vi "Get Modification Flags.vi"(8 "error in (no error)":errorcluster, 10 "Saved VI in":refnum<class "Item.lvclass">, 11 "VI in":refnum<class "VI.lvclass">) -> (0 "error out":errorcluster, 1 "Modification Flags":bool[](array[boolean]), 2 "Saved VI out":refnum<class "VI.lvclass">, 3 "VI out":refnum<class "VI.lvclass">)   [LabVIEW 2020, in "VI Properties Editor.lvlib" / "VI.lvclass"]
doc: "Gets the modification flags of <B>VI in</B> by comparing it to <B>Saved VI in</B>."
uses:
  VI.lvclass
  Item/Item.lvclass
  Control/Control.lvclass
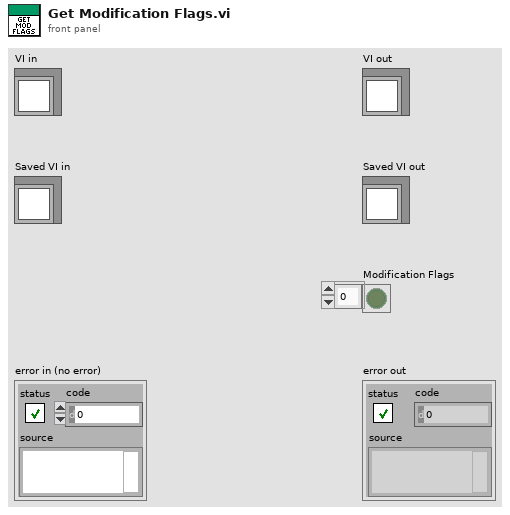
[diagram p1: front panel]
types:
  T1 = enum16{"Share clones between instances", "Preallocate clone for each instance"}
  T2 = enum32{"invalid execution system", "user interface", "standard", "instrument i/o", "data acquisition", "other 1", "other 2", "same as caller"}
  T3 = enum32{"invalid priority", "background priority", "normal priority", "above normal priority", "high priority", "time critical priority", "subroutine"}
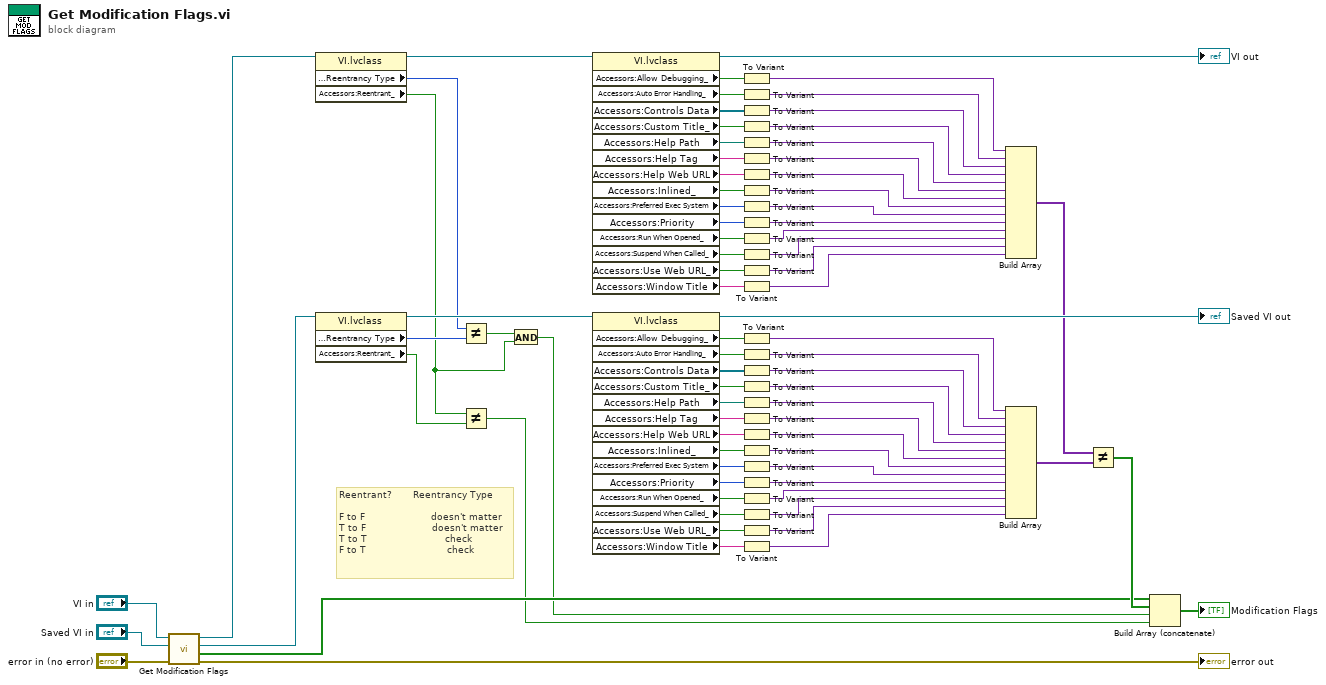
[diagram p0: block diagram]
diagram:
  # "Reentrant?       Reentrancy Type\n\nF to F                      doesn't matter\nT to F                      doesn't matter\nT to T                          check\nF to T                           check"
  n1 = call-parent "Get Modification Flags.vi"("error in (no error)"="error in (no error)", "Saved Item in"="Saved VI in", "Item in"="VI in") -> ("error out"=→"error out":errorcluster, "Modification Flags"=w13:bool[], "Saved Item out"=w10:refnum<class "VI.lvclass">, "Item out"=w8:refnum<class "VI.lvclass">)  [unwired: 5 in]
  n2 = property class="VI.lvclass"(reference=w8) -> (reference out=w9:refnum<class "VI.lvclass">, "Accessors:Reentrancy Type"=w7:T1, "Accessors:Reentrant_"=w1:bool)  [unwired: 1 in, 1 out]
  n3 = property class="VI.lvclass"(reference=w10) -> (reference out=w11:refnum<class "VI.lvclass">, "Accessors:Reentrancy Type"=w6:T1, "Accessors:Reentrant_"=w4:bool)  [unwired: 1 in, 1 out]
  n4 = Not Equal?(x=w7, y=w6) -> (x != y?=w5:bool)
  n5 = Not Equal?(x=w1, y=w4) -> (x != y?=w2:bool)
  n6 = And(x=w5, y=w1) -> (x .and. y?=w3:bool)
  n7 = property class="VI.lvclass"(reference=w9) -> (reference out=→"VI out":refnum<class "VI.lvclass">, "Accessors:Allow Debugging_"=w72:bool, "Accessors:Auto Error Handling_"=w71:bool, "Accessors:Controls Data"=w70:refnum<class "Control.lvclass">[], "Accessors:Custom Title_"=w69:bool, "Accessors:Help Path"=w68:path, "Accessors:Help Tag"=w67:string, "Accessors:Help Web URL"=w66:string, "Accessors:Inlined_"=w65:bool, "Accessors:Preferred Exec System"=w64:T2, "Accessors:Priority"=w63:T3, "Accessors:Run When Opened_"=w62:bool, "Accessors:Suspend When Called_"=w61:bool, "Accessors:Use Web URL_"=w60:bool, "Accessors:Window Title"=w59:string)  [unwired: 1 in, 1 out]
  n8 = property class="VI.lvclass"(reference=w11) -> (reference out=→"Saved VI out":refnum<class "VI.lvclass">, "Accessors:Allow Debugging_"=w16:bool, "Accessors:Auto Error Handling_"=w17:bool, "Accessors:Controls Data"=w18:refnum<class "Control.lvclass">[], "Accessors:Custom Title_"=w19:bool, "Accessors:Help Path"=w20:path, "Accessors:Help Tag"=w21:string, "Accessors:Help Web URL"=w22:string, "Accessors:Inlined_"=w23:bool, "Accessors:Preferred Exec System"=w24:T2, "Accessors:Priority"=w25:T3, "Accessors:Run When Opened_"=w26:bool, "Accessors:Suspend When Called_"=w27:bool, "Accessors:Use Web URL_"=w28:bool, "Accessors:Window Title"=w29:string)  [unwired: 1 in, 1 out]
  n9 = To Variant(anything=w72) -> (Variant=w58:variant)
  n10 = To Variant(anything=w71) -> (Variant=w57:variant)
  n11 = To Variant(anything=w70) -> (Variant=w56:variant)
  n12 = To Variant(anything=w69) -> (Variant=w55:variant)
  n13 = To Variant(anything=w68) -> (Variant=w54:variant)
  n14 = To Variant(anything=w67) -> (Variant=w53:variant)
  n15 = To Variant(anything=w66) -> (Variant=w52:variant)
  n16 = To Variant(anything=w65) -> (Variant=w51:variant)
  n17 = To Variant(anything=w64) -> (Variant=w50:variant)
  n18 = To Variant(anything=w63) -> (Variant=w49:variant)
  n19 = To Variant(anything=w62) -> (Variant=w48:variant)
  n20 = To Variant(anything=w61) -> (Variant=w47:variant)
  n21 = To Variant(anything=w60) -> (Variant=w46:variant)
  n22 = To Variant(anything=w59) -> (Variant=w45:variant)
  n23 = To Variant(anything=w16) -> (Variant=w30:variant)
  n24 = To Variant(anything=w17) -> (Variant=w31:variant)
  n25 = To Variant(anything=w18) -> (Variant=w32:variant)
  n26 = To Variant(anything=w19) -> (Variant=w33:variant)
  n27 = To Variant(anything=w20) -> (Variant=w34:variant)
  n28 = To Variant(anything=w21) -> (Variant=w35:variant)
  n29 = To Variant(anything=w22) -> (Variant=w36:variant)
  n30 = To Variant(anything=w23) -> (Variant=w37:variant)
  n31 = To Variant(anything=w24) -> (Variant=w38:variant)
  n32 = To Variant(anything=w25) -> (Variant=w39:variant)
  n33 = To Variant(anything=w26) -> (Variant=w40:variant)
  n34 = To Variant(anything=w27) -> (Variant=w41:variant)
  n35 = To Variant(anything=w28) -> (Variant=w42:variant)
  n36 = To Variant(anything=w29) -> (Variant=w43:variant)
  n37 = Build Array(w58, w57, w56, w55, w54, w53, w52, w51, w50, w49, w48, w47, w46, w45) -> (w44:variant[])
  n38 = Build Array(w30, w31, w32, w33, w34, w35, w36, w37, w38, w39, w40, w41, w42, w43) -> (w15:variant[])
  n39 = Not Equal?(x=w44, y=w15) -> (x != y?=w14:bool[])
  n40 = Build Array (concatenate)(w13, w14, w3, w2) -> (→"Modification Flags":bool[])
